vi "VM Error Code Description.vi"(6 "extra msg":string, 7 "VC Handle":T1=-1, 9 "VarMan Engine error":T2 items=["No error", "Invalid variable type", "Variable not found", "Variable already exists", "Invalid context handle", "Input error", "Invalid data format", "No history attached", "History already attached", "Invalid history parameters", "Wrong variable name", "Wrong alias name", "Non-unique alias", "Alias not found", "No alias associated", "Alias already associated", "Wrong context name", "Non-unique context name", "Context name not found", "Invalid parameter", "Generic error", "Memory Full", "Unrecognized LV error", "Unknown error code"], 10 "show name spec (F)":bool, 11 "name spec":string) -> (1 "error description":string, 2 "VM VI error code":i32, 3 "error ?":bool)   [LabVIEW 2021]
doc: "::: CalcExpress Toolkit :::\nCopyright (c) 2000-2026 Konstantin Shifershteyn. All rights reserved."
uses:
  cetypes.llb/VarMan Error Code.ctl
  cetypes.llb/VarMan Variable Context Handle.ctl
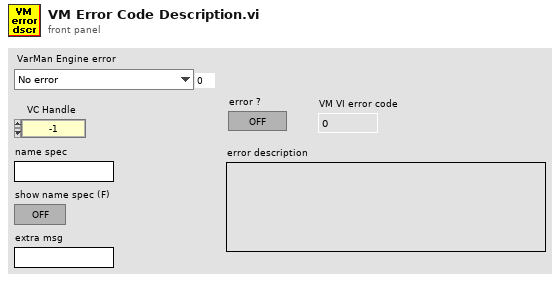
[diagram p1: front panel]
types:
  T1 = typedef "VarMan Variable Context Handle.ctl" = i32
  T2 = typedef "VarMan Error Code.ctl" = u16
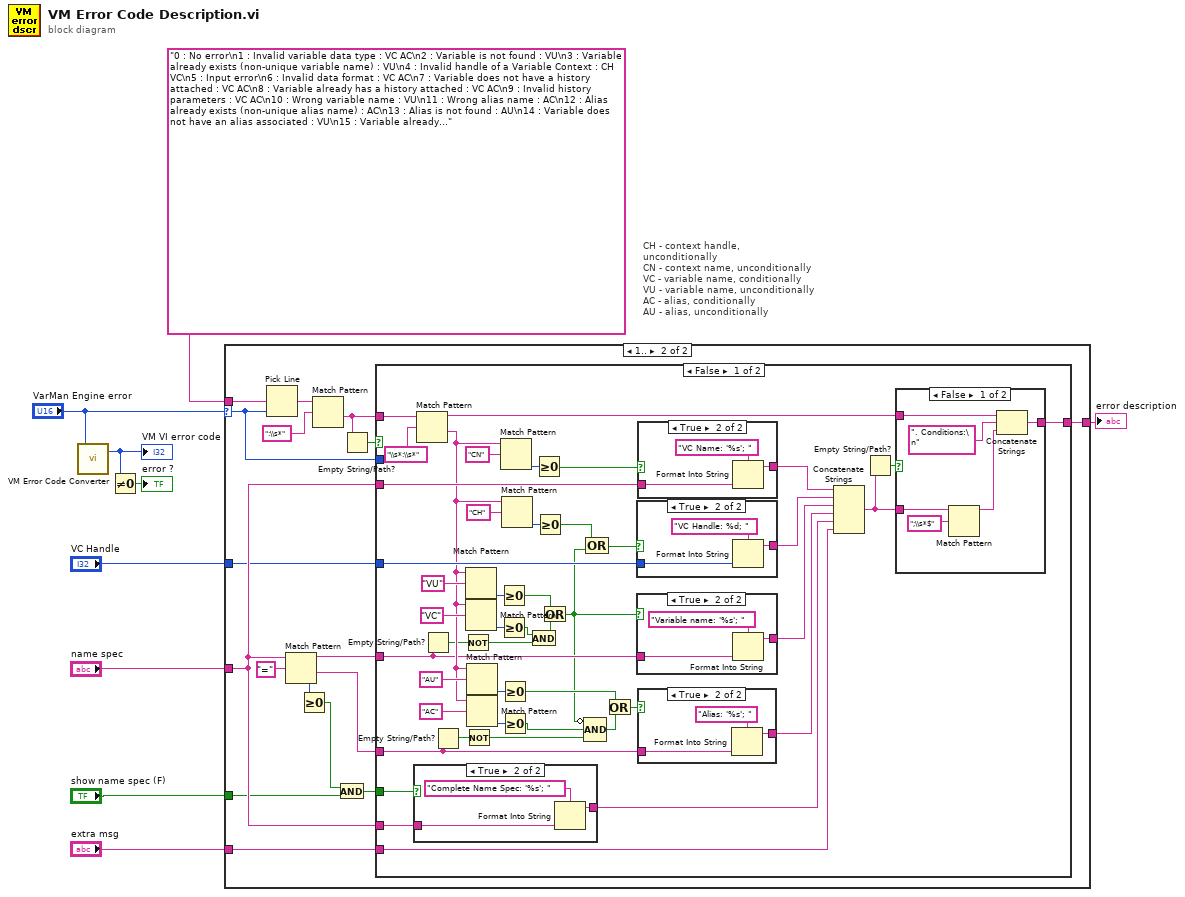
[diagram p0: block diagram]
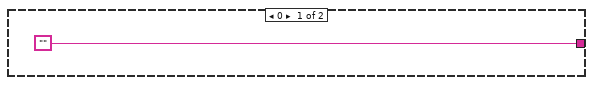
[diagram p2: hidden frame]
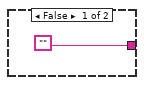
[diagram p3: hidden frame]
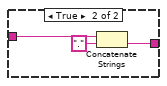
[diagram p4: hidden frame]
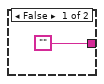
[diagram p5: hidden frame]
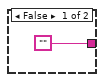
[diagram p6: hidden frame]
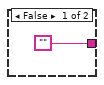
[diagram p7: hidden frame]
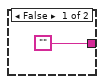
[diagram p8: hidden frame]
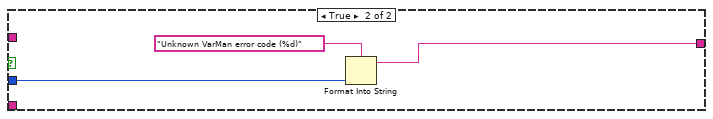
[diagram p9: hidden frame]
diagram:
  # "CH - context handle, unconditionally\nCN - context name, unconditionally\nVC - variable name, conditionally\nVU - variable name, unconditionally\nAC - alias, conditionally\nAU - alias, unconditionally"
  n1 = call "VM Error Code Converter.vi"("VM Engine error code in"="VarMan Engine error") -> ("VM VI error code out"=w3:i32)  [unwired: 1 in, 1 out]
  "VM VI error code" <- w3
  n2 = Not Equal To 0?(x=w3) -> (x != 0?=→"error ?":bool)
  n3 = case shown="1.." "VarMan Engine error" {
    selector: "VarMan Engine error" -> [_ w11]
    tunnel: ["" ("Empty String Constant") w23] -> w9
    tunnel: "0 : No error\n1 : Invalid variable data type : VC AC\n2 : Variable is not found : VU\n3 : Variable already exists (non-unique variable name) : VU\n4 : Invalid handle of a Variable Context : CH VC\n5 : Input error\n6 : Invalid data format : VC AC\n7 : Variable does not have a history attached : VC AC\n8 : Variable already has a history attached : VC AC\n9 : Invalid history parameters : VC AC\n10 : Wrong variable name : VU\n11 : Wrong alias name : AC\n12 : Alias already exists (non-unique alias name) : AC\n13 : Alias is not found : AU\n14 : Variable does not have an alias associated : VU\n15 : Variable already has an alias associated : VU AC\n16 : Wrong context name : CN\n17 : Non-unique context name : CN\n18 : Context name is not found : CN\n19 : Invalid parameters (generic)\n20 : Generic VarMan error\n21 : Memory Full\n22 : Unrecognized LabVIEW manager error" -> [_ w22]
    tunnel: "name spec" -> [_ w18]
    tunnel: "VC Handle" -> [_ w17]
    tunnel: "show name spec (F)" -> [_ w13]
    tunnel: "extra msg" -> [_ w12]
    frame 0 {
    }
    frame 1.. {
      n4 = Pick Line(multi-line string=w22, line index=w11) -> (output string=w27:string)  [unwired: 1 in]
      n5 = Match Pattern(string=w18, regular expression="=") -> (before substring=w20:string, after substring=w19:string, offset past match=w16:i32)  [unwired: 1 in, 1 out]
      n6 = Greater Or Equal To 0?(x=w16) -> (x >= 0?=w15:bool)
      n7 = Match Pattern(string=w27, regular expression=":\\s*") -> (after substring=w24:string)  [unwired: 1 in, 3 out]
      n8 = And(x=w15, y=w13) -> (x .and. y?=w14:bool)
      n9 = Empty String/Path?(string/path=w24) -> (empty?=w25:bool)
      n10 = case shown="False" w25 {
        tunnel: w24 -> [w72 _]
        tunnel: w18 -> [w62 _]
        tunnel: w17 -> [w49 _]
        tunnel: w19 -> [w50 _]
        tunnel: [w58 w103] -> w23
        tunnel: w20 -> [w36 _]
        tunnel: w18 -> [w31 _]
        tunnel: w14 -> [w30 _]
        tunnel: w12 -> [w28 _]
        tunnel: w11 -> [_ w104]
        frame False {
          n11 = case shown="True" w30 {
            tunnel: ["" ("Empty String Constant") w76] -> w32
            tunnel: w31 -> [_ w75]
            frame False {
            }
            frame True {
              n12 = Format Into String(format string="Complete Name Spec: '%s'; ", w75) -> (resulting string=w76:string)  [unwired: 2 in, 1 out]
            }
          }
          n13 = Match Pattern(string=w72, regular expression="\\s*:\\s*") -> (before substring=w59:string, after substring=w45:string)  [unwired: 1 in, 2 out]
          n14 = Empty String/Path?(string/path=w36) -> (empty?=w44:bool)
          n15 = Empty String/Path?(string/path=w50) -> (empty?=w51:bool)
          n16 = Not(x=w44) -> (.not. x?=w43:bool)
          n17 = Not(x=w51) -> (.not. x?=w52:bool)
          n18 = Match Pattern(string=w45, regular expression="VU") -> (offset past match=w47:i32)  [unwired: 1 in, 3 out]
          n19 = Match Pattern(string=w45, regular expression="VC") -> (offset past match=w65:i32)  [unwired: 1 in, 3 out]
          n20 = Match Pattern(string=w45, regular expression="AU") -> (offset past match=w38:i32)  [unwired: 1 in, 3 out]
          n21 = Match Pattern(string=w45, regular expression="AC") -> (offset past match=w64:i32)  [unwired: 1 in, 3 out]
          n22 = Greater Or Equal To 0?(x=w47) -> (x >= 0?=w40:bool)
          n23 = Greater Or Equal To 0?(x=w65) -> (x >= 0?=w41:bool)
          n24 = Greater Or Equal To 0?(x=w38) -> (x >= 0?=w37:bool)
          n25 = Greater Or Equal To 0?(x=w64) -> (x >= 0?=w53:bool)
          n26 = Match Pattern(string=w45, regular expression="CN") -> (offset past match=w67:i32)  [unwired: 1 in, 3 out]
          n27 = Match Pattern(string=w45, regular expression="CH") -> (offset past match=w66:i32)  [unwired: 1 in, 3 out]
          n28 = And(x=w41, y=w43) -> (x .and. y?=w42:bool)
          n29 = Greater Or Equal To 0?(x=w67) -> (x >= 0?=w63:bool)
          n30 = Greater Or Equal To 0?(x=w66) -> (x >= 0?=w34:bool)
          n31 = Or(x=w40, y=w42) -> (x .or. y?=w29:bool)
          n32 = Compound Arithmetic op=AND(invert w29, w53, w52) -> (w39:bool)
          n33 = Compound Arithmetic op=OR(w34, w29) -> (w35:bool)
          n34 = Or(x=w37, y=w39) -> (x .or. y?=w33:bool)
          n35 = case shown="True" w35 {
            tunnel: ["" ("Empty String Constant") w101] -> w56
            tunnel: w49 -> [_ w100]
            frame False {
            }
            frame True {
              n36 = Format Into String(format string="VC Handle: %d; ", w100) -> (resulting string=w101:string)  [unwired: 2 in, 1 out]
            }
          }
          n37 = case shown="True" w29 {
            tunnel: ["" ("Empty String Constant") w97] -> w61
            tunnel: w36 -> [_ w96]
            frame False {
            }
            frame True {
              n38 = Format Into String(format string="Variable name: '%s'; ", w96) -> (resulting string=w97:string)  [unwired: 2 in, 1 out]
            }
          }
          n39 = case shown="True" w63 {
            tunnel: ["" ("Empty String Constant") w89] -> w57
            tunnel: w62 -> [_ w88]
            frame False {
            }
            frame True {
              n40 = Format Into String(format string="VC Name: '%s'; ", w88) -> (resulting string=w89:string)  [unwired: 2 in, 1 out]
            }
          }
          n41 = case shown="True" w33 {
            tunnel: ["" ("Empty String Constant") w93] -> w55
            tunnel: w50 -> [_ w92]
            frame False {
            }
            frame True {
              n42 = Format Into String(format string="Alias: '%s'; ", w92) -> (resulting string=w93:string)  [unwired: 2 in, 1 out]
            }
          }
          n43 = Concatenate Strings(w57, w56, w61, w55, w32, w28) -> (w54:string)
          n44 = Empty String/Path?(string/path=w54) -> (empty?=w60:bool)
          n45 = case shown="False" w60 {
            tunnel: w59 -> [w83 w86]
            tunnel: w54 -> [w80 _]
            tunnel: [w81 w84] -> w58
            frame False {
              n46 = Match Pattern(string=w80, regular expression=";\\s*$") -> (before substring=w78:string)  [unwired: 1 in, 3 out]
              n47 = Concatenate Strings(w83, ". Conditions:\n", w78) -> (w81:string)
            }
            frame True {
              n48 = Concatenate Strings(w86, ".") -> (w84:string)
            }
          }
        }
        frame True {
          n49 = Format Into String(format string="Unknown VarMan error code (%d)", w104) -> (resulting string=w103:string)  [unwired: 2 in, 1 out]
        }
      }
    }
  }
  "error description" <- w9
